vi "Find OOB Server Ports.vi"(8 "error in":errorcluster) -> (3 "Ports":u16[](array[numeric]))   [LabVIEW 2025]
uses:
  <vilib>/Utility/error.llb/Trim Whitespace One-Sided.vi
panel:
  out "return code":i32
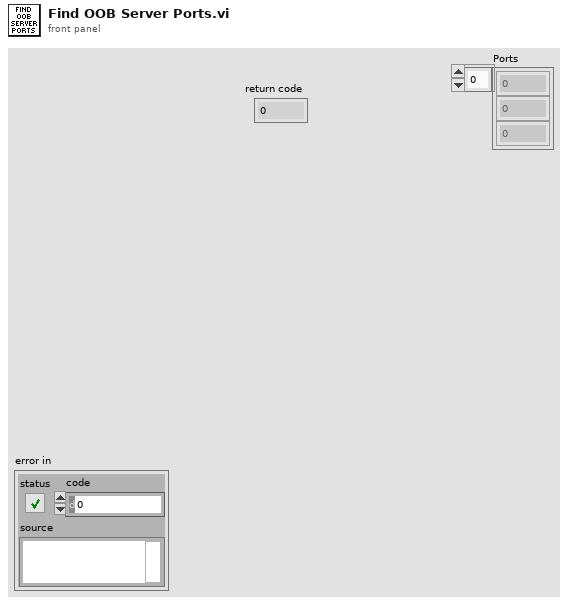
[diagram p1: front panel]
types:
  T1 = cluster{"Protocol":enum16{"invalid", "tcp", "udp", "icmp", "ip", "tcpv6", "udpv6", "icmpv6", "ipv6"}, "LocalIP":string, "LocalPort":u16, "ForeignIP":string, "ForeignPort":u16, "State":enum8{"UNKNOWN", "LISTEN", "ESTABLISHED", "SYN_SENT", "SYN_RECV", "LAST_ACK", "CLOSE_WAIT", "TIME_WAIT", "CLOSED", "CLOSING", "FIN_WAIT1", "FIN_WAIT2"}, "PID":u16}[]
  T2 = enum8{"UNKNOWN", "LISTEN", "ESTABLISHED", "SYN_SENT", "SYN_RECV", "LAST_ACK", "CLOSE_WAIT", "TIME_WAIT", "CLOSED", "CLOSING", "FIN_WAIT1", "FIN_WAIT2"}
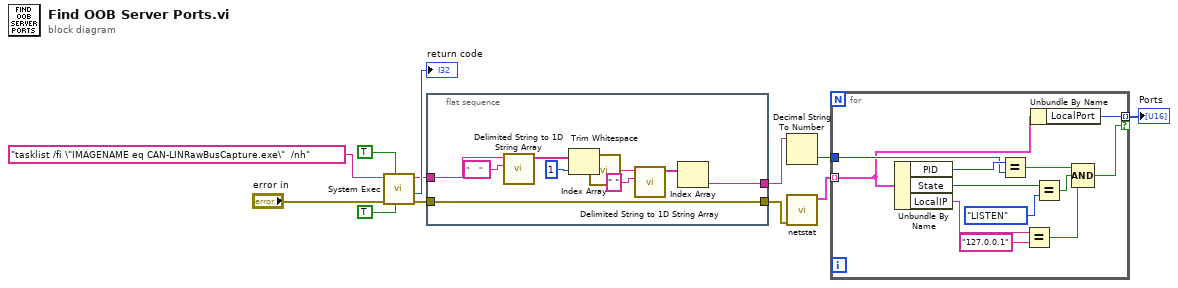
[diagram p0: block diagram]
diagram:
  n1 = call <vilib>:"System Exec.vi"("run minimized? (F)"=TRUE, "wait until completion? (T)"=TRUE, "error in (no error)"="error in", "command line"="tasklist /fi \"IMAGENAME eq CAN-LINRawBusCapture.exe\"  /nh") -> ("error out"=w7:errorcluster, "return code"=→"return code":i32, "standard output"=w5:string)  [unwired: 4 in, 1 out]
  n2 = flat-sequence {
    tunnel: w5 -> [w22]
    tunnel: [w15] -> w6
    tunnel: w7 -> [w14]
    tunnel: [w14] -> w2
    frame #0 {
      n3 = call <vilib>:"Delimited String to 1D String Array.vi"("delimiter"="     ", "delimited string"=w22) -> ("string array"=w20:string[])  [unwired: 9 in]
      n4 = Index Array(array=w20, index=1) -> (element=w18:string)
      n5 = call <vilib>:"Trim Whitespace.vi"("string"=w18) -> ("trimmed string"=w13:string)  [unwired: 1 in]
      n6 = call <vilib>:"Delimited String to 1D String Array.vi"("delimiter"=" ", "delimited string"=w13) -> ("string array"=w16:string[])  [unwired: 9 in]
      n7 = Index Array(array=w16) -> (element=w15:string)  [unwired: 1 in]
    }
  }
  n8 = Decimal String To Number(string=w6) -> (number=w4:i32)  [unwired: 2 in, 1 out]
  n9 = call "netstat.vi"("error in (no error)"=w2) -> ("netstat"=w3:T1)  [unwired: 9 in, 1 out]
  n10 = for {
    tunnel: w3 -> [w25] mode=indexing
    tunnel: w4 -> [w33]
    tunnel: [w24] -> w1 mode=indexing if=w23
    n11 = Unbundle By Name(w25) -> ("PID"=w34:u16, "State"=w31:T2, "LocalIP"=w28:string)
    n12 = Equal?(x=w34, y=w33) -> (x = y?=w32:bool)
    n13 = Equal?(x=w28, y="127.0.0.1") -> (x = y?=w26:bool)
    n14 = Unbundle By Name(w25) -> ("LocalPort"=w24:u16)
    n15 = Equal?(x=w31, y=T2."LISTEN") -> (x = y?=w29:bool)
    n16 = Compound Arithmetic op=AND(w32, w29, w26) -> (w23:bool)
  }
  "Ports" <- w1
